vi "python_vi.vi"() -> ()   [LabVIEW 2025]
panel:
  out "String 2":string
  in  "String":string
  in  "stop":bool
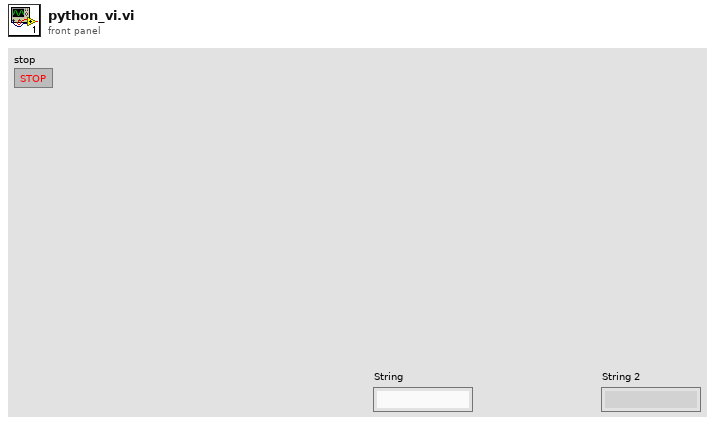
[diagram p1: front panel]
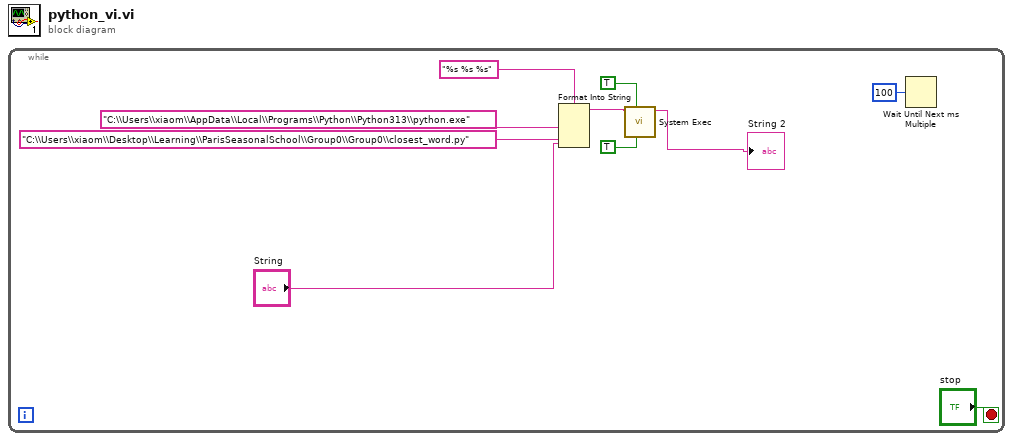
[diagram p0: block diagram]
diagram:
  n1 = while {
    stop <- "stop" stop-if-true
    n2 = Format Into String(format string="%s %s %s", "C:\\Users\\xiaom\\AppData\\Local\\Programs\\Python\\Python313\\python.exe" ("input 6"), "C:\\Users\\xiaom\\Desktop\\Learning\\ParisSeasonalSchool\\Group0\\Group0\\closest_word.py" ("input 6"), "String") -> (resulting string=w5:string)  [unwired: 2 in, 1 out]
    n3 = call <vilib>:"System Exec.vi"("run minimized? (F)"=TRUE, "wait until completion? (T)"=TRUE, "command line"=w5) -> ("standard output"=→"String 2":string)  [unwired: 5 in, 3 out]
    n4 = Wait Until Next ms Multiple(millisecond multiple=u32 100) -> ()  [unwired: 1 out]
  }
